vi "Get value.vi"(0 "Stack in":refnum<class "Stack.lvclass">, 11 "error in (no error)":errorcluster) -> (3 "PUT Settings":T1, 4 "Stack out":refnum<class "Stack.lvclass">, 6 "Resolution Geometry":string, 10 "Assembly Settings":T1, 14 "Component Settings":T1, 15 "error out":errorcluster)   [LabVIEW 2021, in "Stack.lvclass"]
uses:
  Stack.lvclass
  Stack.lvclass/Stack.ctl
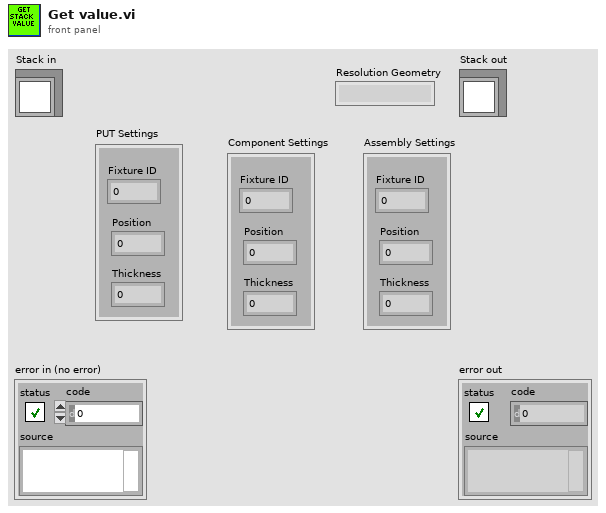
[diagram p1: front panel]
types:
  T1 = cluster{"Fixture ID":dbl, "Position":dbl, "Thickness":dbl}
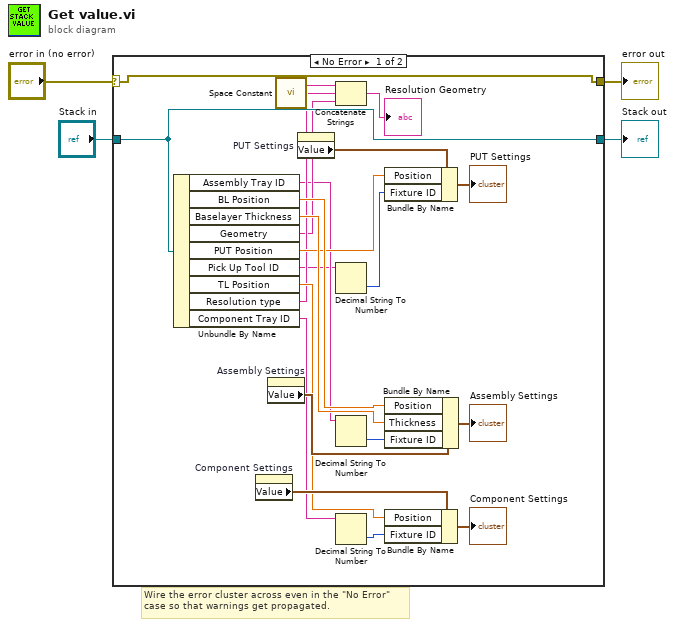
[diagram p0: block diagram]
diagram:
  # "Wire the error cluster across even in the \"No Error\"\ncase so that warnings get propagated."
  n1 = case shown="No Error" "error in (no error)" {
    selector: "error in (no error)" -> [w26 w28]
    tunnel: [w26 w28] -> w3
    tunnel: [w25 w27] -> w1
    tunnel: "Stack in" -> [w25 w27]
    frame No Error {
      n2 = Unbundle By Name(w25) -> ("Assembly Tray ID"=w10:string, "BL Position"=w21:dbl, "Baselayer Thickness"=w22:dbl, "Geometry"=w13:string, "PUT Position"=w16:dbl, "Pick Up Tool ID"=w6:string, "TL Position"=w15:dbl, "Resolution type"=w14:string, "Component Tray ID"=w9:string)
      n3 = property on="Component Settings" class="Clust (strict)"() -> ("Value"=w20:T1)  [unwired: 2 in, 2 out]
      n4 = property on="Assembly Settings" class="Clust (strict)"() -> ("Value"=w23:T1)  [unwired: 2 in, 2 out]
      n5 = call <vilib>:"Space Constant.vi"() -> ("String"=w11:string)
      n6 = property on="PUT Settings" class="Clust (strict)"() -> ("Value"=w18:T1)  [unwired: 2 in, 2 out]
      n7 = Concatenate Strings(w14, w11, w13) -> (→"Resolution Geometry":string)
      n8 = Decimal String To Number(string=w6) -> (number=w7:i32)  [unwired: 2 in, 1 out]
      n9 = Decimal String To Number(string=w10) -> (number=w5:i32)  [unwired: 2 in, 1 out]
      n10 = Decimal String To Number(string=w9) -> (number=w8:i32)  [unwired: 2 in, 1 out]
      n11 = Bundle By Name(cluster=w18, "Position"=w16, "Fixture ID"=w7) -> (→"PUT Settings":T1)
      n12 = Bundle By Name(cluster=w23, "Position"=w21, "Thickness"=w22, "Fixture ID"=w5) -> (→"Assembly Settings":T1)
      n13 = Bundle By Name(cluster=w20, "Position"=w15, "Fixture ID"=w8) -> (→"Component Settings":T1)
    }
    frame Error {
    }
  }
  "error out" <- w3
  "Stack out" <- w1
